vi "Array to Temp.vi"(9 "Temperatures":dbl[](array[numeric])) -> (0 "LHP":cluster{"LH T1":dbl, "LH T2":dbl, "LH T3":dbl}, 1 "UHP":cluster{"UH T1":dbl, "UH T2":dbl, "UH T3":dbl}, 2 "LCP":cluster{"LC T1":dbl, "LC T2":dbl, "LC T3":dbl}, 3 "UCP":cluster{"UC T1":dbl, "UC T2":dbl, "UC T3":dbl}, 4 "Temperatures":dbl[](array[numeric]))   [LabVIEW 2026]
panel:
  in  "Temperatures 2":dbl[](array[numeric])=[6547.3, 6551.3, 1.6, 29.4, 29.0, 29.2, 30.8, 30.7, 24.7, 23.8, 18.7]
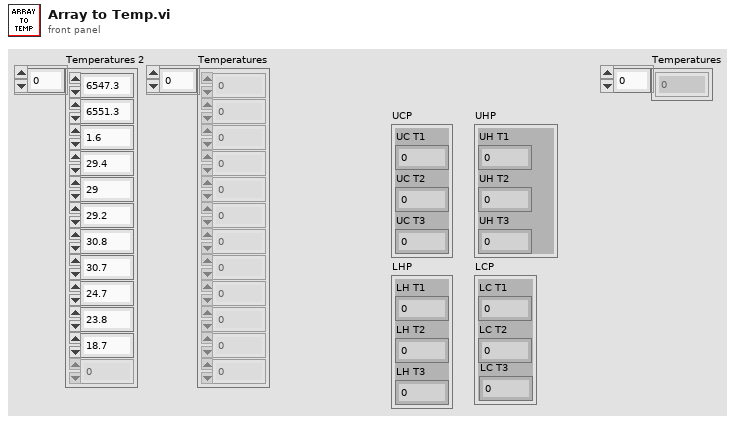
[diagram p1: front panel]
types:
  T1 = cluster{"Temperatures":dbl, "Temperatures":dbl, "Temperatures":dbl}
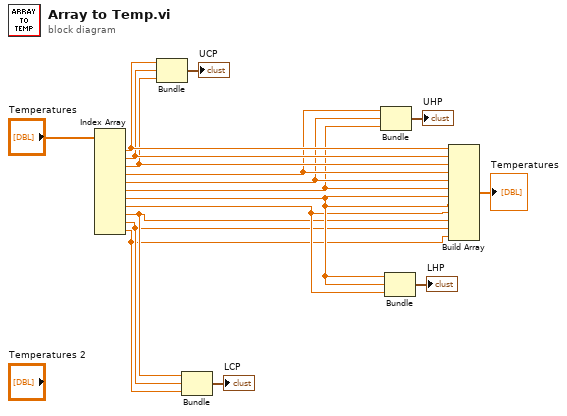
[diagram p0: block diagram]
diagram:
  n1 = Index Array(array="Temperatures") -> (element #1=w14:dbl, element #2=w13:dbl, element #3=w12:dbl, element #4=w11:dbl, element #5=w10:dbl, element #6=w9:dbl, element #7=w5:dbl, element #8=w4:dbl, element #9=w3:dbl, element #10=w2:dbl, element #11=w1:dbl)  [unwired: 11 in]
  n2 = Bundle("Temperatures"=w14, "Temperatures"=w13, "Temperatures"=w12) -> (→"UCP":T1)  [unwired: 1 in]
  n3 = Bundle("Temperatures"=w3, "Temperatures"=w2, "Temperatures"=w1) -> (→"LCP":T1)  [unwired: 1 in]
  n4 = Bundle("Temperatures"=w11, "Temperatures"=w10, "Temperatures"=w9) -> (→"UHP":T1)  [unwired: 1 in]
  n5 = Bundle("Temperatures"=w5, "Temperatures"=w5, "Temperatures"=w4) -> (→"LHP":T1)  [unwired: 1 in]
  n6 = Build Array(w14, w13, w12, w11, w10, w9, w5, w5, w4, w3, w2, w1) -> (→"Temperatures":dbl[])
